vi "5001 Mismatch Parameter Count.vi"(8 "error in (no error)":errorcluster, 11 "Parameter Count":i32) -> (0 "error out":errorcluster)   [LabVIEW 2020, in "VI Properties Editor.lvlib" / "Custom Errors.lvlib"]
uses:
  Custom Errors.lvlib
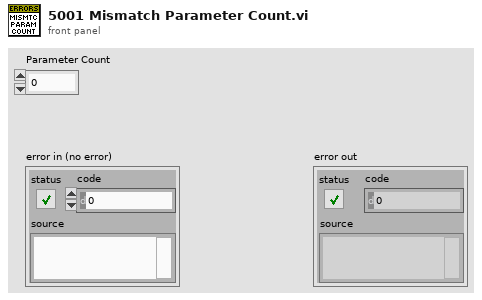
[diagram p1: front panel]
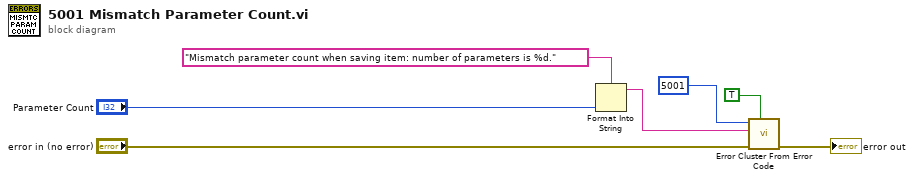
[diagram p0: block diagram]
diagram:
  n1 = Format Into String(format string="Mismatch parameter count when saving item: number of parameters is %d.", "Parameter Count") -> (resulting string=w3:string)  [unwired: 2 in, 1 out]
  n2 = call <vilib>:"Error Cluster From Error Code.vi"("show call chain? (False)"=TRUE, "error in (no error)"="error in (no error)", "error message (\"\")"=w3, "error code (0)"=5001) -> ("error out"=→"error out":errorcluster)  [unwired: 5 in]
